vi "Set.vi"(6 "Labels":map{string, string}(c390), 8 "error in (no error)":errorcluster, 10 "Value":dbl, 11 "Gauge Ref":refnum<data-value>) -> (0 "error out":errorcluster, 3 "Gauge Ref out":refnum<data-value>)   [LabVIEW 2020, in "Metrics.lvlib" / "Gauge.lvclass"]
doc: "Sets the value of the gauge to the value passed as Value parameter."
uses:
  Gauge.lvclass
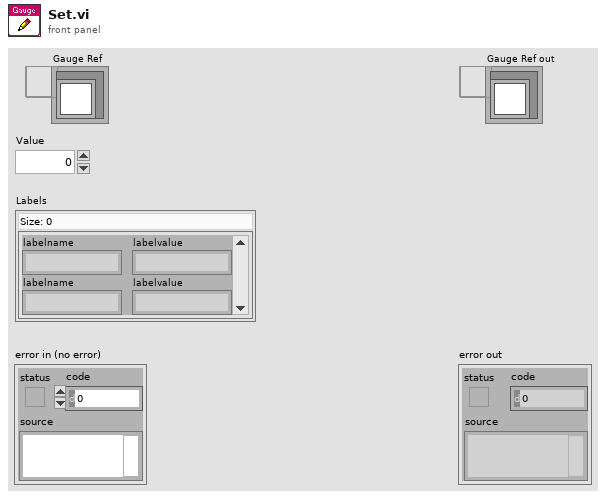
[diagram p1: front panel]
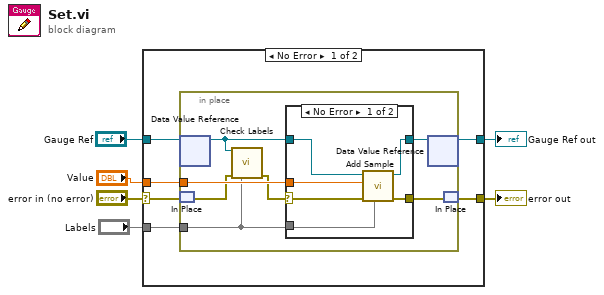
[diagram p0: block diagram]
diagram:
  n1 = case shown="No Error" "error in (no error)" {
    selector: "error in (no error)" -> [w8 w28]
    tunnel: [w7 w28] -> w5
    tunnel: "Gauge Ref" -> [w12 _]
    tunnel: "Value" -> [w11 _]
    tunnel: "Labels" -> [w10 _]
    tunnel: [w9 _] -> w1
    frame No Error {
      n2 = in-place {
        in-place-border: w11 -> [w19]
        in-place-border: w10 -> [w15]
        n3 = in-place-dvr #1(w12) -> (w16:refnum<class "Gauge.lvclass">)  [unwired: 1 out]
        n4 = in-place-match #2(w8) -> (w14:errorcluster)
        n5 = call-dynamic "Check Labels.vi"("Metric in"=w16, "error in (no error)"=w14, "Labels"=w15) -> ("error out"=w13:errorcluster)  [unwired: 9 in, 3 out]
        n6 = case shown="No Error" w13 {
          selector: w13 -> [w23 w26]
          tunnel: w19 -> [w25 _]
          tunnel: [w24 w27] -> w18
          tunnel: [w22 w26] -> w17
          tunnel: w16 -> [w21 w27]
          tunnel: w15 -> [w20 _]
          frame No Error {
            n7 = call-dynamic "Add Sample.vi"("Labels"=w20, "error in (no error)"=w23, "Value"=w25, "Metric in"=w21) -> ("error out"=w22:errorcluster, "Metric out"=w24:refnum<class "Gauge.lvclass">)  [unwired: 6 in]
          }
          frame Error {
          }
        }
        n8 = in-place-dvr #1(w18) -> (w9:refnum<data-value>)  [unwired: 1 out]
        n9 = in-place-match #2(w17) -> (w7:errorcluster)
      }
    }
    frame Error {
    }
  }
  "error out" <- w5
  "Gauge Ref out" <- w1
